vi "Resize Panes.vi"(8 "error in (no error)":errorcluster caption="错误输入（无错误）", 11 "Data Viewer 输入":refnum<class "Data Viewer.lvclass">) -> (0 "error out":errorcluster caption="错误输出", 3 "Data Viewer 输出":refnum<class "Data Viewer.lvclass">)   [LabVIEW 2020, in "Data Viewer.lvlib" / "Data Viewer.lvclass"]
uses:
  Data Viewer.lvclass
  <vilib>/Utility/miscctls.llb/LVPointTypeDef.ctl
  <vilib>/Utility/miscctls.llb/LVRectTypeDef.ctl
  <vilib>/Utility/miscctls.llb/LVForegroundBackgroundColorsTypeDef.ctl
  Data Viewer.lvclass/Data Viewer.ctl
  Data Viewer.lvlib
panel:
  out "map":map{i32, u32}(c390)
  out "Right Width":u32
  out "left":u32
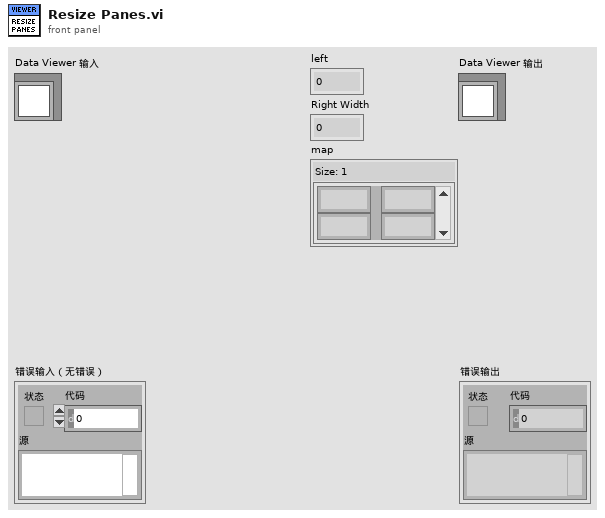
[diagram p1: front panel]
types:
  T1 = typedef "LVForegroundBackgroundColorsTypeDef.ctl" = cluster{"Foreground Color":u32, "Background Color":u32}
  T2 = typedef "LVRectTypeDef.ctl" = cluster{"Left":i16, "Top":i16, "Right":i16, "Bottom":i16}
  T3 = typedef "LVPointTypeDef.ctl" = cluster{"Horizontal":i16, "Vertical":i16}
  T4 = typedef "LVPositionTypeDef.ctl" = cluster{"Left":i32, "Top":i32}
  T5 = typedef "LVBoundsTypeDef.ctl" = cluster{"Width":u32, "Height":u32}
  T6 = typedef "DataSave.lvlib/Data Viewer.lvlib/Data Viewer.lvclass/Legend.ctl" = cluster{"颜色":u32, "曲线名称":string}[]
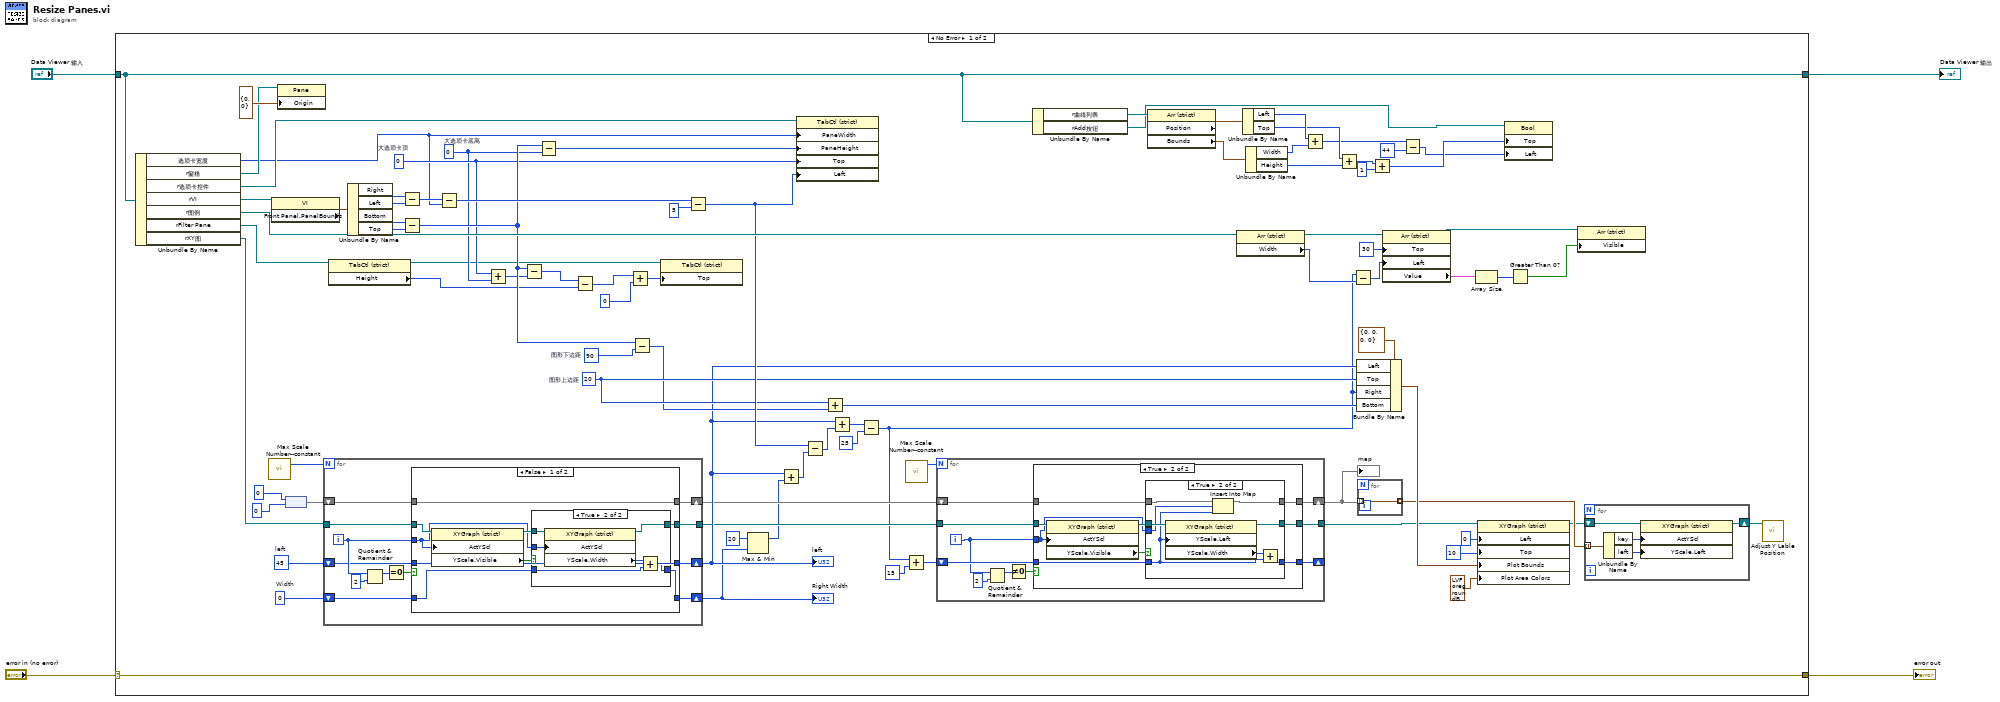
[diagram p0: block diagram]
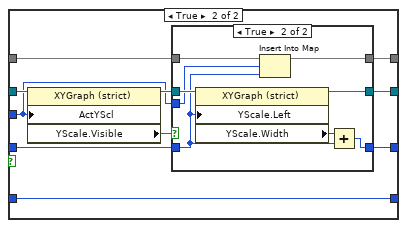
[diagram p5: hidden frame]
diagram:
  n1 = case shown="No Error" "error in (no error)" {
    selector: "error in (no error)" -> [w90 w181]
    tunnel: [w90 w181] -> w3
    tunnel: [w24 w180] -> w1
    tunnel: "Data Viewer 输入" -> [w24 w180]
    frame No Error {
      w48 = 0  # Width
      w50 = 45  # left
      w54 = i16 20  # 图形上边距
      w66 = i16 0  # 大选项卡底高
      w79 = i16 90  # 图形下边距
      w67 = 0  # 大选项卡顶
      n2 = Unbundle By Name(w24) -> ("选项卡宽度"=w27:u32, "r窗格"=w29:refnum<vi>, "r选项卡控件"=w28:refnum<vi>, "rVI"=w86:refnum<vi>, "r图例"=w77:refnum<vi>, "rFilter Pane"=w65:refnum<vi>, "rXY图"=w26:refnum<vi>)
      n3 = call "Max Scale Number--constant.vi"() -> ("Max Scale Number"=w51:i32)  [unwired: 11 in]
      n4 = property class="VI"(reference=w86) -> ("Front Panel.PanelBounds"=w85:T2)  [unwired: 1 in, 2 out]
      n5 = property class="Pane"(reference=w29, "Origin"=T3 {"Horizontal"=0, "Vertical"=0} ("原点")) -> ()  [unwired: 1 in, 2 out]
      n6 = node(0, u32 0 ("left")) -> (w43:map{i32, u32})
      n7 = for {
        N: w51 -> [_]
        tunnel: w26 -> [w138]
        shift-right: [w135] -> w49
        shift-left: w50 -> [w136]
        shift-right: [w133] -> w33
        shift-left: w48 -> [w134]
        shift-right: [w131] -> w42
        shift-left: w43 -> [w132]
        tunnel: [w130] -> w38
        i -> [w137]
        n8 = Quotient & Remainder(x=w137, y=2) -> (x-y*floor(x/y)=w140:i32)  [unwired: 1 out]
        n9 = Equal To 0?(x=w140) -> (x = 0?=w139:bool)
        n10 = case shown="False" w139 {
          tunnel: w138 -> [w147 w168]
          tunnel: w137 -> [w144 w162]
          tunnel: w136 -> [w150 w165]
          tunnel: [w150 w164] -> w135
          tunnel: w134 -> [w146 w163]
          tunnel: [w145 w163] -> w133
          tunnel: w132 -> [w143 w161]
          tunnel: [w143 w160] -> w131
          tunnel: [w142 w159] -> w130
          frame False {
            n11 = property class="XYGraph (strict)"(reference=w147, "ActYScl"=w144) -> (reference out=w148:refnum<vi>, "YScale.Visible"=w149:bool)  [unwired: 1 in, 1 out]
            n12 = case shown="True" w149 {
              tunnel: w148 -> [w151 w158]
              tunnel: w146 -> [w152 w157]
              tunnel: [w152 w156] -> w145
              tunnel: w144 -> [_ w154]
              tunnel: [w151 w153] -> w142
              frame False {
              }
              frame True {
                n13 = property class="XYGraph (strict)"(reference=w158, "ActYScl"=w154) -> (reference out=w153:refnum<vi>, "YScale.Width"=w155:u32)  [unwired: 1 in, 1 out]
                n14 = Add(x=w155, y=w157) -> (x+y=w156:u32)
              }
            }
          }
          frame True {
            n15 = property class="XYGraph (strict)"(reference=w168, "ActYScl"=w162) -> (reference out=w166:refnum<vi>, "YScale.Visible"=w167:bool)  [unwired: 1 in, 1 out]
            n16 = case shown="True" w167 {
              tunnel: w166 -> [w169 w179]
              tunnel: w165 -> [w171 w174]
              tunnel: [w171 w177] -> w164
              tunnel: w162 -> [_ w175]
              tunnel: w161 -> [w170 w176]
              tunnel: [w170 w173] -> w160
              tunnel: [w169 w172] -> w159
              frame False {
              }
              frame True {
                n17 = property class="XYGraph (strict)"(reference=w179, "YScale.Left"=w174) -> (reference out=w172:refnum<vi>, "YScale.Width"=w178:u32)  [unwired: 1 in, 1 out]
                n18 = Insert Into Map(map in=w176, key=w175, value=w174) -> (map out=w173:map{i32, u32})  [unwired: 2 out]
                n19 = Add(x=w178, y=w174) -> (x+y=w177:u32)
              }
            }
          }
        }
      }
      "left" <- w49
      "Right Width" <- w33
      n20 = property class="TabCtl (strict)"(reference=w65) -> (reference out=w64:refnum<vi>, "Height"=w61:u32)  [unwired: 1 in, 1 out]
      n21 = Unbundle By Name(w85) -> ("Right"=w84:i16, "Left"=w83:i16, "Bottom"=w81:i16, "Top"=w80:i16)
      n22 = Subtract(x=w84, y=w83) -> (x-y=w82:i16)
      n23 = Subtract(x=w81, y=w80) -> (x-y=w68:i16)
      n24 = Subtract(x=w82, y=w27) -> (x-y=w89:u32)
      n25 = Add(x=w67, y=w66) -> (x+y=w63:i32)
      n26 = Subtract(x=w68, y=w63) -> (x-y=w62:i32)
      n27 = Subtract(x=w68, y=w66) -> (x-y=w69:i16)
      n28 = Subtract(x=w62, y=w61) -> (x-y=w60:u32)
      n29 = Add(x=w60, y=u32 0) -> (x+y=w59:u32)
      n30 = Subtract(x=w68, y=w79) -> (x-y=w53:i16)
      n31 = property class="TabCtl (strict)"(reference=w64, "Top"=w59) -> ()  [unwired: 1 in, 2 out]
      n32 = Subtract(x=w89, y=u32 5) -> (x-y=w72:u32)
      n33 = Max & Min(x=u32 20 ("y"), y=w33) -> (max(x,y)=w36:u32)  [unwired: 1 out]
      n34 = Add(x=w49, y=w36) -> (x+y=w71:u32)
      n35 = property class="TabCtl (strict)"(reference=w28, "PaneWidth"=w27, "PaneHeight"=w69, "Top"=w67, "Left"=w72) -> ()  [unwired: 1 in, 2 out]
      n36 = Subtract(x=w72, y=w71) -> (x-y=w55:u32)
      n37 = Add(x=w54, y=w53) -> (x+y=w52:i16)
      n38 = Add(x=w49, y=w55) -> (x+y=w39:u32)
      n39 = Subtract(x=w39, y=u32 25) -> (x-y=w8:u32)
      n40 = Add(x=w8, y=u32 15 ("x")) -> (x+y=w37:u32)
      n41 = call "Max Scale Number--constant.vi"() -> ("Max Scale Number"=w47:i32)  [unwired: 11 in]
      n42 = for {
        N: w47 -> [_]
        shift-right: [w102] -> _
        shift-left: w37 -> [w103]
        tunnel: w38 -> [w101]
        shift-right: [w98] -> w41
        shift-left: w42 -> [w99]
        tunnel: [w97] -> w31
        i -> [w100]
        n43 = Quotient & Remainder(x=w100, y=2) -> (x-y*floor(x/y)=w105:i32)  [unwired: 1 out]
        n44 = Not Equal To 0?(x=w105) -> (x != 0?=w104:bool)
        n45 = case shown="True" w104 {
          tunnel: w100 -> [_ w113]
          tunnel: w103 -> [w109 w116]
          tunnel: [w109 w115] -> w102
          tunnel: w101 -> [w107 w114]
          tunnel: w99 -> [w108 w112]
          tunnel: [w108 w111] -> w98
          tunnel: [w107 w110] -> w97
          frame False {
          }
          frame True {
            n46 = property class="XYGraph (strict)"(reference=w114, "ActYScl"=w113) -> (reference out=w117:refnum<vi>, "YScale.Visible"=w118:bool)  [unwired: 1 in, 1 out]
            n47 = case shown="True" w118 {
              tunnel: w117 -> [w119 w129]
              tunnel: w116 -> [w121 w124]
              tunnel: [w121 w127] -> w115
              tunnel: w113 -> [_ w125]
              tunnel: w112 -> [w120 w126]
              tunnel: [w120 w123] -> w111
              tunnel: [w119 w122] -> w110
              frame False {
              }
              frame True {
                n48 = property class="XYGraph (strict)"(reference=w129, "YScale.Left"=w124) -> (reference out=w122:refnum<vi>, "YScale.Width"=w128:u32)  [unwired: 1 in, 1 out]
                n49 = Insert Into Map(map in=w126, key=w125, value=w124) -> (map out=w123:map{i32, u32})  [unwired: 2 out]
                n50 = Add(x=w128, y=w124) -> (x+y=w127:u32)
              }
            }
          }
        }
      }
      "map" <- w41
      n51 = Unbundle By Name(w24) -> ("r曲线列表"=w23:refnum<vi>, "rAdd按钮"=w14:refnum<vi>)
      n52 = property class="Arr (strict)"(reference=w23) -> ("Position"=w22:T4, "Bounds"=w21:T5)  [unwired: 1 in, 2 out]
      n53 = property class="Arr (strict)"(reference=w77) -> (reference out=w76:refnum<vi>, "Width"=w74:u32)  [unwired: 1 in, 1 out]
      n54 = Unbundle By Name(w22) -> ("Left"=w19:i32, "Top"=w18:i32)
      n55 = Unbundle By Name(w21) -> ("Width"=w20:u32, "Height"=w17:u32)
      n56 = Add(x=w19, y=w20) -> (x+y=w12:u32)
      n57 = Add(x=w18, y=w17) -> (x+y=w16:u32)
      n58 = Subtract(x=w8, y=w74) -> (x-y=w73:u32)
      n59 = Bundle By Name(cluster=T2 {"Left"=0, "Top"=0, "Right"=0, "Bottom"=0} ("Plot Area Bounds"), "Left"=w49, "Top"=w54, "Right"=w8, "Bottom"=w52) -> (w56:T2)
      n60 = for {
        tunnel: [w91] -> w40 mode=indexing
        tunnel: w41 -> [w91] mode=indexing
      }
      n61 = Add(x=w16, y=u32 1) -> (x+y=w13:u32)
      n62 = property class="Arr (strict)"(reference=w76, "Top"=30 ("位置:置顶"), "Left"=w73) -> (reference out=w9:refnum<vi>, "Value"=w7:T6)  [unwired: 1 in, 1 out]
      n63 = Subtract(x=w12, y=u32 44) -> (x-y=w10:u32)
      n64 = Array Size(array=w7) -> (size(s)=w6:i32)
      n65 = property class="XYGraph (strict)"(reference=w31, "Left"=0 ("位置:居左"), "Top"=10 ("位置:置顶"), "Plot Bounds"=w56, "Plot Area Colors"=T1 {"Foreground Color"=9868950, "Background Color"=16777216} ("Plot Area:Colors")) -> (reference out=w30:refnum<vi>)  [unwired: 1 in, 1 out]
      n66 = property class="Bool"(reference=w14, "Top"=w13, "Left"=w10) -> ()  [unwired: 1 in, 2 out]
      n67 = Greater Than 0?(x=w6) -> (x > 0?=w5:bool)
      n68 = property class="Arr (strict)"(reference=w9, "Visible"=w5) -> ()  [unwired: 1 in, 2 out]
      n69 = for {
        shift-right: [w95] -> w32
        shift-left: w30 -> [w96]
        tunnel: w40 -> [w94] mode=indexing
        n70 = Unbundle By Name(w94) -> ("key"=w93:i32, "left"=w92:u32)
        n71 = property class="XYGraph (strict)"(reference=w96, "ActYScl"=w93, "YScale.Left"=w92) -> (reference out=w95:refnum<vi>)  [unwired: 1 in, 1 out]
      }
      n72 = call "Adjust Y Lable Position.vi"("XY图 2"=w32) -> ()  [unwired: 11 in]
    }
    frame Error {
    }
  }
  "error out" <- w3
  "Data Viewer 输出" <- w1
